vi "test access allowed clients.vi"(8 "error in (no error)":errorcluster) -> (0 "error out":errorcluster, 3 "body":string)   [LabVIEW 2020, in "MCP Server tests.lvlib"]
doc: "Client allow-list. A second MCP server is started on port 37061 with Allowed clients = [\"192.0.2.1\"] (TEST-NET-1, never this computer). A tools/list from this computer is refused before any MCP handling: HTTP 403, Content-Type application/json and the JSON-RPC error {\"jsonrpc\":\"2.0\",\"id\":null,\"error\":{\"code\":-32600,\"message\":\"Forbidden: client not allowed.\"}}. The server is stopped afterwards. That the default (empty Allowed clients) still lets this computer in is shown by every other test."
uses:
  MCP Server tests.lvlib
  <vilib>/addons/_JKI Toolkits/Caraya/classes/Test/Test.lvclass
  src/MCP Server/MCP Server.lvlib
  <vilib>/addons/_JKI Toolkits/Caraya/classes/Assert/Assert.lvclass
panel:
  out "lookup error":errorcluster
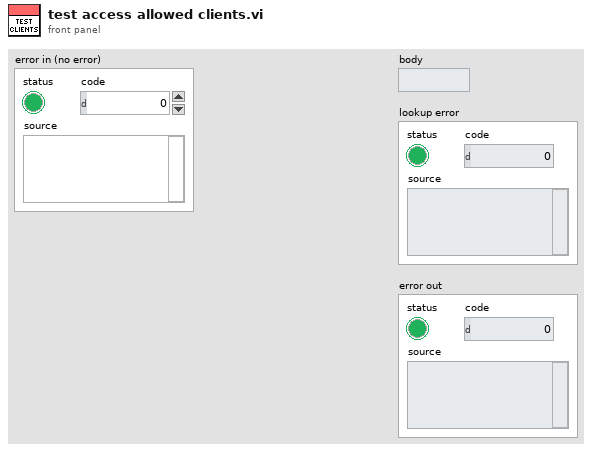
[diagram p1: front panel]
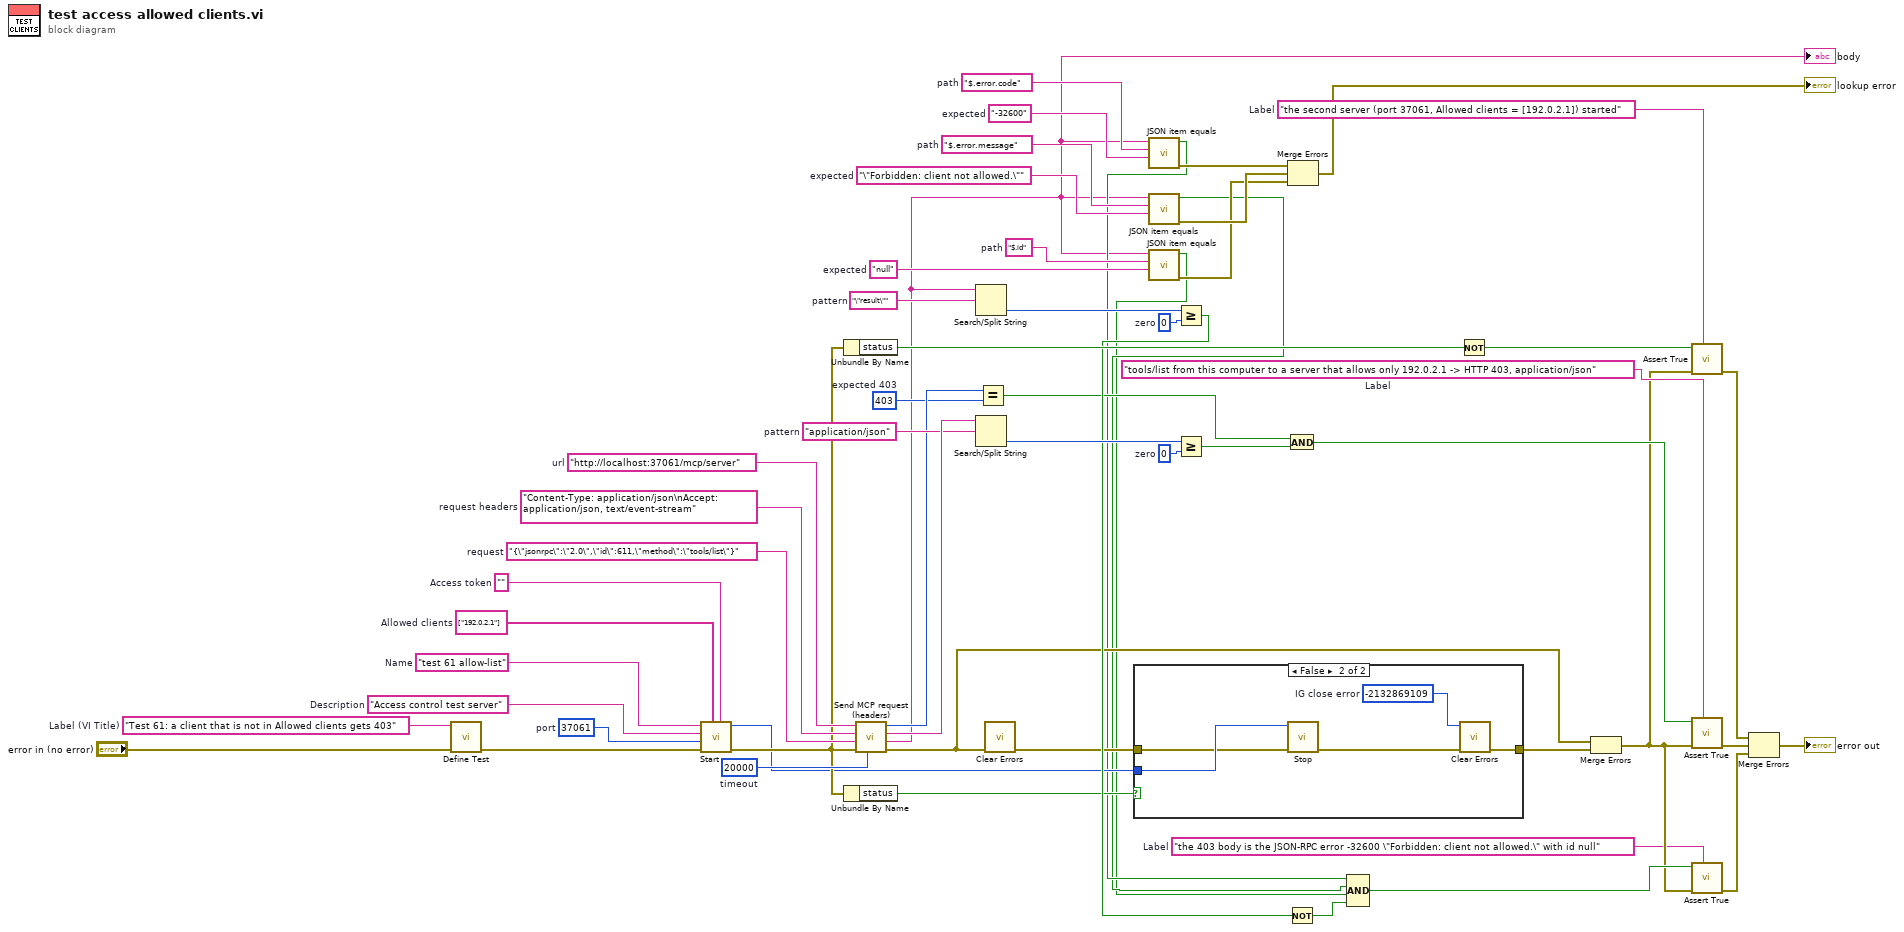
[diagram p0: block diagram]
diagram:
  w47 = "Content-Type: application/json\nAccept: application/json, text/event-stream"  # request headers
  w7 = "the 403 body is the JSON-RPC error -32600 \"Forbidden: client not allowed.\" with id null"  # Label
  w10 = "tools/list from this computer to a server that allows only 192.0.2.1 -> HTTP 403, application/json"  # Label
  w12 = "the second server (port 37061, Allowed clients = [192.0.2.1]) started"  # Label
  w28 = 0  # zero
  w41 = "\"result\""  # pattern
  w31 = "null"  # expected
  w32 = "$.id"  # path
  w35 = "\"Forbidden: client not allowed.\""  # expected
  w36 = "$.error.message"  # path
  w37 = "-32600"  # expected
  w38 = "$.error.code"  # path
  w39 = 0  # zero
  w42 = "application/json"  # pattern
  w26 = 403  # expected 403
  w45 = 20000  # timeout
  w46 = "{\"jsonrpc\":\"2.0\",\"id\":611,\"method\":\"tools/list\"}"  # request
  w48 = "http://localhost:37061/mcp/server"  # url
  w50 = ""  # Access token
  w51 = string[] ["192.0.2.1"]  # Allowed clients
  w53 = u16 37061  # port
  w54 = "Access control test server"  # Description
  w55 = "test 61 allow-list"  # Name
  w57 = "Test 61: a client that is not in Allowed clients gets 403"  # Label (VI Title)
  n1 = call <vilib>:"Define Test.vi"("error in (no error)"="error in (no error)", "Label (VI Title)"=w57) -> ("error out"=w52:errorcluster)  [unwired: 8 in, 1 out]
  n2 = call "Start.vi"("Access token"=w50, "Allowed clients"=w51, "error in (no error)"=w52, "HTTP Port (36987)"=w53, "Description"=w54, "Name"=w55) -> ("error out"=w44:errorcluster, "server id out"=w24:i32)  [unwired: 3 in, 1 out]
  n3 = Unbundle By Name(w44) -> ("status"=w49:bool)
  n4 = Unbundle By Name(w44) -> ("status"=w22:bool)
  n5 = call "Send MCP request (headers).vi"("timeout (10000)"=w45, "error in (no error)"=w44, "request"=w46, "request headers"=w47, "url"=w48) -> ("error out"=w19:errorcluster, "response"=w3:string, "headers"=w43:string, "status code"=w27:i32)  [unwired: 3 in]
  "body" <- w3
  n6 = Search/Split String(string=w3, search string/char (-)=w41) -> (offset of match=w29:i32)  [unwired: 1 in, 2 out]
  n7 = Search/Split String(string=w43, search string/char (-)=w42) -> (offset of match=w40:i32)  [unwired: 1 in, 2 out]
  n8 = Equal?(x=w27, y=w26) -> (x = y?=w21:bool)
  n9 = call <vilib>:"Clear Errors.vi"("error in (no error)"=w19) -> ("error out"=w23:errorcluster)  [unwired: 5 in, 1 out]
  n10 = case shown="False" w22 {
    tunnel: w24 -> [_ w63]
    tunnel: w23 -> [w58 w62]
    tunnel: [w58 w59] -> w18
    frame True {
    }
    frame False {
      w61 = -2132869109  # IG close error
      n11 = call "Stop.vi"("error in (no error)"=w62, "id"=w63) -> ("error out"=w60:errorcluster)  [unwired: 9 in]
      n12 = call <vilib>:"Clear Errors.vi"("error in (no error)"=w60, "specific error code to clear (0: all)"=w61) -> ("error out"=w59:errorcluster)  [unwired: 4 in, 1 out]
    }
  }
  n13 = call "JSON item equals.vi"("expected"=w37, "path"=w38, "JSON"=w3) -> ("error out"=w34:errorcluster, "equal?"=w17:bool)  [unwired: 6 in, 1 out]
  n14 = call "JSON item equals.vi"("expected"=w35, "path"=w36, "JSON"=w3) -> ("error out"=w33:errorcluster, "equal?"=w16:bool)  [unwired: 6 in, 1 out]
  n15 = call "JSON item equals.vi"("expected"=w31, "path"=w32, "JSON"=w3) -> ("error out"=w30:errorcluster, "equal?"=w15:bool)  [unwired: 6 in, 1 out]
  n16 = Greater Or Equal?(x=w29, y=w28) -> (x >= y?=w25:bool)
  n17 = Greater Or Equal?(x=w40, y=w39) -> (x >= y?=w20:bool)
  n18 = And(x=w21, y=w20) -> (x .and. y?=w11:bool)
  n19 = Not(x=w25) -> (.not. x?=w14:bool)
  n20 = Merge Errors(w34, w33, w30) -> (→"lookup error":errorcluster)
  n21 = Compound Arithmetic op=AND(w17, w16, w15, w14) -> (w9:bool)
  n22 = Not(x=w49) -> (.not. x?=w13:bool)
  n23 = Merge Errors(w19, w18) -> (w8:errorcluster)
  n24 = call <vilib>:"Assert True.vi"("Label"=w12, "error in (no error)"=w8, "True?"=w13) -> ("error out"=w6:errorcluster)  [unwired: 7 in, 1 out]
  n25 = call <vilib>:"Assert True.vi"("Label"=w10, "error in (no error)"=w8, "True?"=w11) -> ("error out"=w5:errorcluster)  [unwired: 7 in, 1 out]
  n26 = call <vilib>:"Assert True.vi"("Label"=w7, "error in (no error)"=w8, "True?"=w9) -> ("error out"=w4:errorcluster)  [unwired: 7 in, 1 out]
  n27 = Merge Errors(w6, w5, w4) -> (→"error out":errorcluster)
